vi "Origen User Events.vi"() -> ()   [LabVIEW 2026]
panel:
  in  "stop":bool
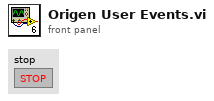
[diagram p1: front panel]
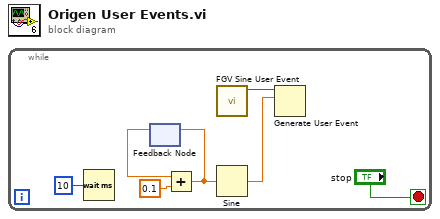
[diagram p0: block diagram]
diagram:
  n1 = while {
    stop <- "stop" stop-if-true
    n2 = Wait (ms)(milliseconds to wait=u32 10) -> ()  [unwired: 1 out]
    n3 = feedback #1() -> (w6:dbl)  [unwired: 1 in]
    n4 = Add(x=w6, y=0.1) -> (x+y=w5:dbl)
    n5 = feedback-in #1(w5) -> ()
    n6 = call "FGV Sine User Event.vi"() -> ("User Event out"=w1:refnum<user-event>)  [unwired: 10 in, 1 out]
    n7 = Sine(x=w5) -> (sin(x)=w7:dbl)
    n8 = Generate User Event(user event=w1, event data cluster=w7) -> ()  [unwired: 2 in, 2 out]
  }
